vi "Dispense.vi"(8 "error in (no error)":errorcluster, 11 "Dispenser In":refnum<visa-resource-name>) -> (0 "error out":errorcluster, 3 "Dispenser Out":refnum<visa-resource-name>)   [LabVIEW 2020, in "Ultimus V.lvclass"]
uses:
  Ultimus V.lvclass
  Drivers/EFD Ultimus V/EFD Ultimus V.lvlib
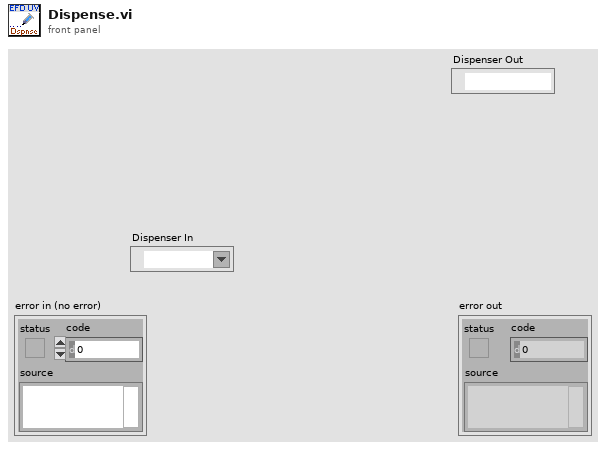
[diagram p1: front panel]
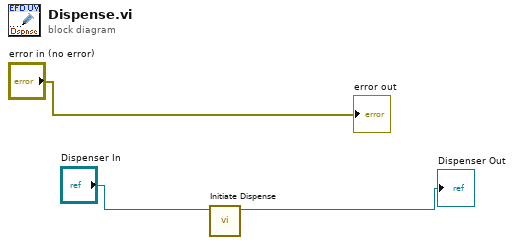
[diagram p0: block diagram]
diagram:
  n1 = call "Initiate Dispense.vi"("VISA resource name"="Dispenser In") -> ("VISA resource name out"=→"Dispenser Out":refnum<visa-resource-name>)  [unwired: 9 in, 1 out]
  "error out" <- "error in (no error)"
